vi "View Packages and Package Attributes.vi"() -> ()   [LabVIEW 2014]
doc: "This example shows how to list installed/available/upgradable packages and view a package's attributes."
uses:
  NIPM_API.lvlib
panel:
  in  "Tab Control":T1(tab)
  out "Upgradable packages":string[][](table)
  out "Installed packages":string[][](table)
  out "Available packages to install":string[][](table)
  in  "List packages?":bool
  out "Package found?":bool
  in  "Get package attributes?":bool
  in  "Package name":string
  in  "Version":string
  out "Package attributes":string[][](table)
  # "1. On the List Packages tab, set the List packages control to TRUE to get a list of installed, available, and upgradable packages.\n2. On the Get Attributes of a Package tab, set the Get package attributes control to TRUE and specify a Package name and Version to get the package's attributes.\n3. Run this VI."
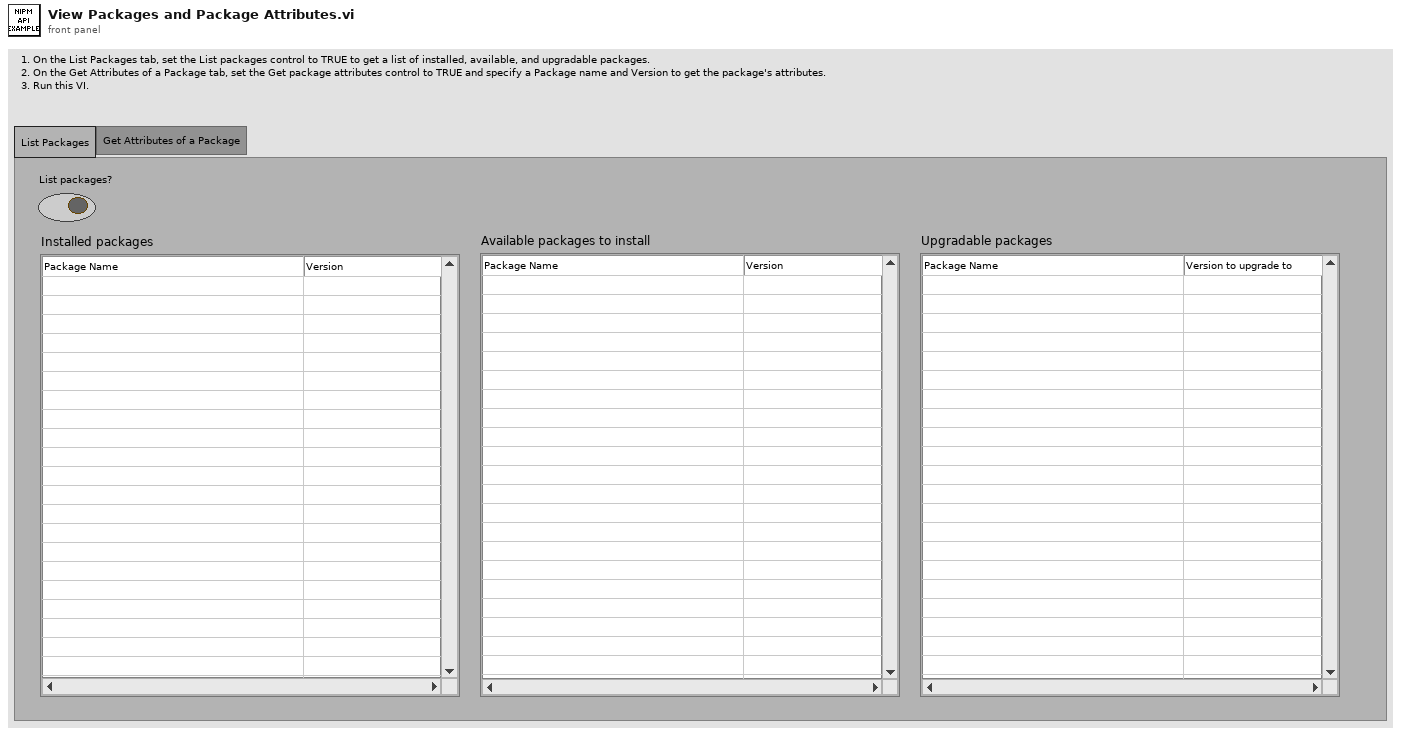
[diagram p1: front panel]
types:
  T1 = enum32{"List Packages", "Get Attributes of a Package"}
  T2 = typedef "NIPM_API.lvlib/package attributes.ctl" = cluster{"Package Name":string, "Display name":string, "Version":string, "Display version":string, "Synopsis":string, "Description":string, "Maintainer":string, "Maintainer email address":string, "Category":string, "Homepage":string, "Release notes":string, "Depends":string[], "Recommends":string[], "Suggests":string[], "Conflicts":string[], "Provides":string[], "Replaces":string[], "Supplements":string[], "Enhances":string[], "Product":bool, "User visible":bool, "Installed size (KB)":u64, "Package filesize (bytes)":u64, "Architecture":string, "Agent":string, "MD5Checksum":string}
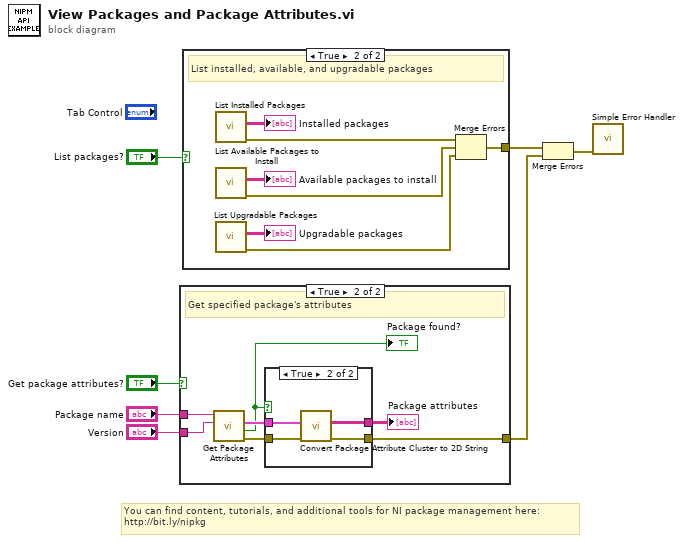
[diagram p0: block diagram]
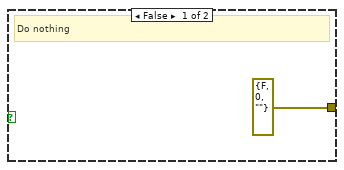
[diagram p2: hidden frame]
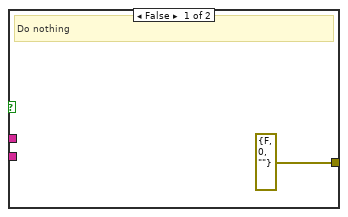
[diagram p3: hidden frame]
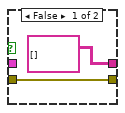
[diagram p4: hidden frame]
diagram:
  # "You can find content, tutorials, and additional tools for NI package management here:\nhttp://bit.ly/nipkg"
  n1 = case shown="True" "Get package attributes?" {
    tunnel: "Package name" -> [_ w15]
    tunnel: "Version" -> [_ w14]
    tunnel: [errorcluster {"status"=FALSE, "code"=0, "source"=""} ("error IO") w11] -> w1
    frame False {
      # "Do nothing"
    }
    frame True {
      # "Get specified package's attributes"
      n2 = call "Get Package Attributes.vi"("version"=w14, "package name"=w15) -> ("error out"=w12:errorcluster, "found?"=w9:bool, "package attributes"=w13:T2)  [unwired: 6 in, 1 out]
      "Package found?" <- w9
      n3 = case shown="True" w9 {
        tunnel: w13 -> [_ w21]
        tunnel: w12 -> [w17 w20]
        tunnel: [w17 w19] -> w11
        tunnel: [string[][] [] ("package attributes (2D string)") w18] -> w10
        frame False {
        }
        frame True {
          n4 = call "Convert Package Attribute Cluster to 2D String.vi"("error in (no error)"=w20, "package attributes (cluster)"=w21) -> ("error out"=w19:errorcluster, "package attributes (2D string)"=w18:string[][])  [unwired: 8 in]
        }
      }
      "Package attributes" <- w10
    }
  }
  n5 = case shown="True" "List packages?" {
    tunnel: [errorcluster {"status"=FALSE, "code"=0, "source"=""} ("error IO") w24] -> w2
    frame False {
      # "Do nothing"
    }
    frame True {
      # "List installed, available, and upgradable packages"
      n6 = call "List Installed Packages.vi"() -> ("error out"=w27:errorcluster, "installed packages"=→"Installed packages":string[][])  [unwired: 10 in]
      n7 = call "List Available Packages to Install.vi"() -> ("error out"=w26:errorcluster, "available packages to install"=→"Available packages to install":string[][])  [unwired: 10 in]
      n8 = call "List Upgradable Packages.vi"() -> ("error out"=w25:errorcluster, "upgradable packages"=→"Upgradable packages":string[][])  [unwired: 10 in]
      n9 = Merge Errors(w27, w26, w25) -> (w24:errorcluster)
    }
  }
  n10 = Merge Errors(w2, w1) -> (w3:errorcluster)
  n11 = call <vilib>:"Simple Error Handler.vi"("error in (no error)"=w3) -> ()  [unwired: 4 in, 5 out]
